vi "GetNodeMenuOptions.vi"(0 "reference in":refnum<class "DQMHModuleNode.lvclass">, 1 "MousePos":T1 {"y" format="%.2f"; "x" format="%.2f"}, 5 "error in (no error)":errorcluster) -> (14 "reference out":refnum<class "DQMHModuleNode.lvclass">, 15 "MenuOptions":string[](array[string]), 19 "error out":errorcluster)   [LabVIEW 2020, in "DQMHModuleNode.lvclass"]
doc: "Gets the menu option"
uses:
  <resource>/Framework/Providers/Open_GDS/UML/DQMHModuleNode_class/DQMHModuleNode.lvclass
  C:/Program Files (x86)/National Instruments/LabVIEW 2020/resource/Framework/Providers/Open_GDS/UML/RectangularNode_class/RectangularNode.lvclass
  <resource>/Framework/Providers/Open_GDS/UML/General/Point/Point Point2D.ctl
  <resource>/Framework/Providers/Open_GDS/UML/RectangularNode_class/RectangularNode.lvclass
  <resource>/Framework/Providers/Open_GDS/UML/MultiLineString_class/MultiLineString.lvclass
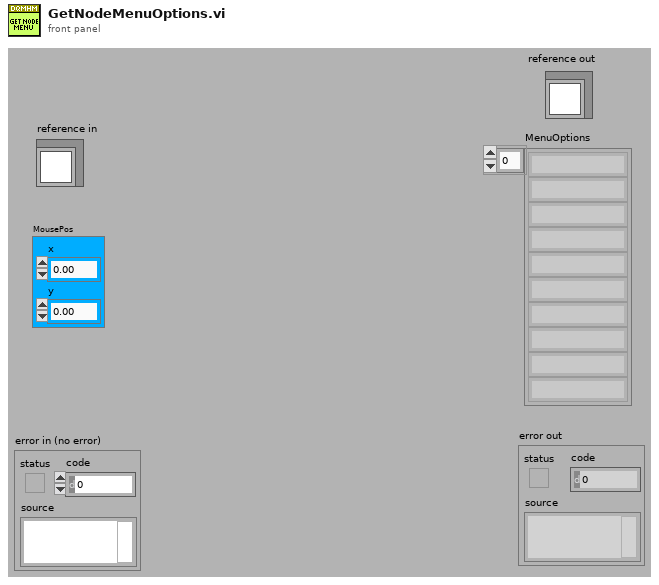
[diagram p1: front panel]
types:
  T1 = typedef "Point Point2D.ctl" = cluster{"x":dbl, "y":dbl}
  T2 = typedef "DQMHModuleNode.lvclass/ObjectAttributes.ctl" = cluster{"DescriptionHeight":dbl, "InternalDataHeight":dbl, "EventsHeight":dbl, "Name":refnum<class "MultiLineString.lvclass">, "Description":refnum<class "MultiLineString.lvclass">, "InternalData":refnum<class "MultiLineString.lvclass">, "Events":refnum<class "MultiLineString.lvclass">, "showDescription":bool, "showInternalData":bool, "showEvents":bool, "DEFAULT_ROUNDING":i32, "DEFAULT_WIDTH":i32, "DEFAULT_HEIGHT":i32, "ClassPath":path, "Template":string, "Icon":u8[][]}
  T3 = typedef "RectangularNode.lvclass/ObjectAttributes.ctl" = cluster{"bounds":T4}
  T4 = typedef "Rectangle Rectangle2D.ctl" = cluster{"x":dbl, "y":dbl, "width":dbl, "height":dbl}
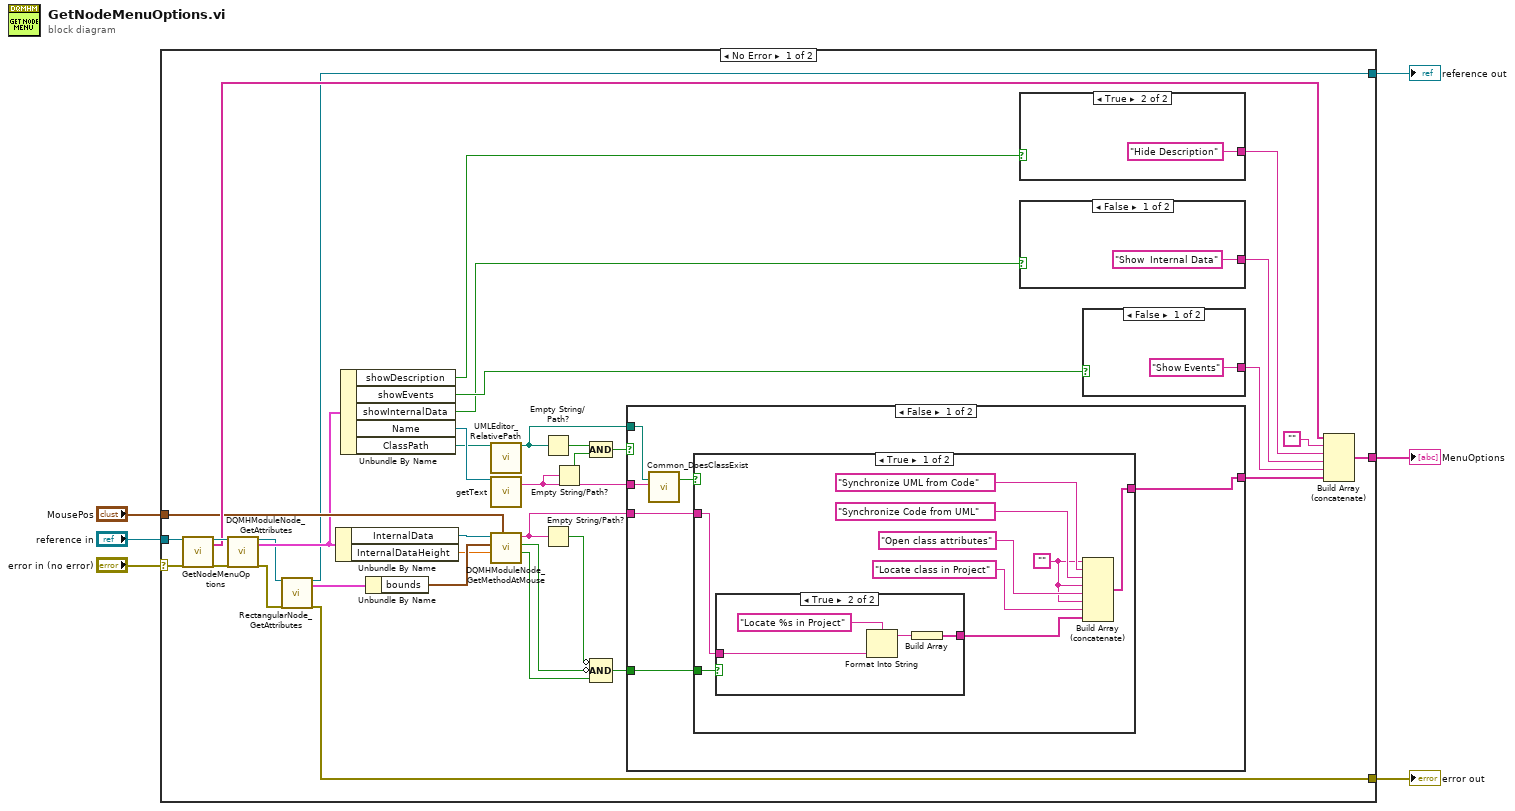
[diagram p0: block diagram]
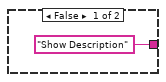
[diagram p2: hidden frame]
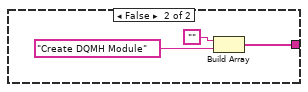
[diagram p4: hidden frame]
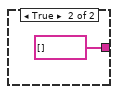
[diagram p5: hidden frame]
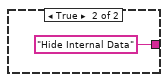
[diagram p6: hidden frame]
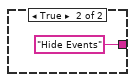
[diagram p7: hidden frame]
diagram:
  n1 = case shown="No Error" "error in (no error)" {
    selector: "error in (no error)" -> [w32 w72]
    tunnel: "reference in" -> [w33 w73]
    tunnel: [w18 w72] -> w5
    tunnel: [w17 w73] -> w4
    tunnel: [w15 _] -> w2
    tunnel: "MousePos" -> [w29 _]
    frame No Error {
      n2 = call-parent "GetNodeMenuOptions.vi"("reference"=w33, "error in (no error)"=w32) -> ("reference out"=w35:refnum<class "DQMHModuleNode.lvclass">, "MenuOptions"=w34:string[], "error out"=w31:errorcluster)  [unwired: 15 in]
      n3 = call <resource>:"DQMHModuleNode_GetAttributes.vi"("reference in"=w35, "error in (no error)"=w31) -> ("reference out"=w20:refnum<class "DQMHModuleNode.lvclass">, "Data"=w21:T2, "error out"=w19:errorcluster)  [unwired: 1 in, 14 out]
      n4 = call <resource>:"RectangularNode_GetAttributes.vi"("reference in"=w20, "error in (no error)"=w19) -> ("reference out"=w17:refnum<class "DQMHModuleNode.lvclass">, "Data"=w16:T3, "error out"=w18:errorcluster)  [unwired: 14 in, 1 out]
      n5 = Unbundle By Name(w21) -> ("InternalData"=w30:refnum<class "MultiLineString.lvclass">, "InternalDataHeight"=w27:dbl)
      n6 = Unbundle By Name(w21) -> ("showDescription"=w14:bool, "showEvents"=w42:bool, "showInternalData"=w41:bool, "Name"=w37:refnum<class "MultiLineString.lvclass">, "ClassPath"=w36:path)
      n7 = Unbundle By Name(w16) -> ("bounds"=w28:T4)
      n8 = call <resource>:"UMLEditor_RelativePath.vi"("Path In"=w36) -> ("ConvertToAbsolutePath(If possible)"=w9:path)  [unwired: 1 in, 17 out]
      n9 = call-dynamic "getText.vi"("reference"=w37) -> ("text"=w8:string)  [unwired: 16 in, 2 out]
      n10 = call <resource>:"DQMHModuleNode_GetMethodAtMouse.vi"("MousePos"=w29, "botHeight"=w27, "bounds"=w28, "reference in"=w30) -> ("MethodSelected"=w25:bool, "NoMmethodsExists"=w26:bool, "MEthodName"=w22:string)  [unwired: 2 in, 1 out]
      n11 = Empty String/Path?(string/path=w9) -> (empty?=w11:bool)
      n12 = Empty String/Path?(string/path=w22) -> (empty?=w24:bool)
      n13 = Empty String/Path?(string/path=w8) -> (empty?=w7:bool)
      n14 = Compound Arithmetic op=AND(w11, w7) -> (w10:bool)
      n15 = Compound Arithmetic op=AND(invert w24, invert w26, w25) -> (w23:bool)
      n16 = case shown="False" w10 {
        tunnel: [w50 string[] []] -> w40
        tunnel: w9 -> [w49 _]
        tunnel: w8 -> [w48 _]
        tunnel: w23 -> [w47 _]
        tunnel: w22 -> [w46 _]
        frame False {
          n17 = call <resource>:"Common_DoesClassExist.vi"("ClassPath"=w49, "ClassName"=w48) -> ("ClassExists"=w45:bool)  [unwired: 17 out]
          n18 = case shown="True" w45 {
            tunnel: [w59 w66] -> w50
            tunnel: w47 -> [w53 _]
            tunnel: w46 -> [w52 _]
            frame True {
              w55 = ""
              n19 = case shown="True" w53 {
                tunnel: w52 -> [_ w63]
                tunnel: [_ w60] -> w51
                frame False {
                }
                frame True {
                  n20 = Format Into String(format string="Locate %s in Project" ("element"), w63) -> (resulting string=w61:string)  [unwired: 2 in, 1 out]
                  n21 = Build Array(w61) -> (w60:string[])
                }
              }
              n22 = Build Array (concatenate)(w55, "Synchronize UML from Code" ("element"), "Synchronize Code from UML" ("element"), w55, "Open class attributes" ("element"), w55, "Locate class in Project" ("element"), w51) -> (w59:string[])
            }
            frame False {
              n23 = Build Array("", "Create DQMH Module" ("element")) -> (w66:string[])
            }
          }
        }
        frame True {
        }
      }
      n24 = case shown="True" w14 {
        tunnel: ["Show Description" "Hide Description"] -> w12
        frame False {
        }
        frame True {
        }
      }
      n25 = case shown="False" w41 {
        tunnel: ["Show  Internal Data" "Hide Internal Data"] -> w38
        frame False {
        }
        frame True {
        }
      }
      n26 = case shown="False" w42 {
        tunnel: ["Show Events" "Hide Events"] -> w39
        frame False {
        }
        frame True {
        }
      }
      n27 = Build Array (concatenate)(w34, "", w12, w38, w39, w40) -> (w15:string[])
    }
    frame Error {
    }
  }
  "reference out" <- w4
  "error out" <- w5
  "MenuOptions" <- w2
